vi "Main_Base.vi"() -> ()   [LabVIEW 2019]
uses:
  <vilib>/myRIO/Common/Instrument Driver Framework/myRIO v1.0/Encoder/typedefs/Encoder Signal Mode.ctl
  <vilib>/myRIO/Common/Instrument Driver Framework/myRIO v1.0/Encoder/typedefs/Encoder Configuration v1.0.ctl
  <vilib>/myRIO/Instrument Drivers/Onboard IO/Encoder/typedefs/Encoder Reference.ctl
  <vilib>/myRIO/Common/Instrument Driver Framework/Utilities/typedefs/myRIO Generic Hardware Reference.ctl
  <vilib>/myRIO/Common/Instrument Driver Framework/Utilities/typedefs/Hardware Version Enum.ctl
  <vilib>/myRIO/Common/Instrument Driver Framework/Utilities/typedefs/myRIO v1.0 Reference.ctl
  <vilib>/myRIO/Common/Instrument Driver Framework/Utilities/typedefs/Generic FPGA Reference.ctl
  <vilib>/myRIO/Common/Instrument Driver Framework/myRIO v1.0/Encoder/typedefs/Encoder Channels Enum.ctl
  <vilib>/userDefined/High Color/nirio_resource_hc.ctl
  <vilib>/myRIO/Instrument Drivers/Onboard IO/DIO/typedefs/DIO Reference.ctl
  <vilib>/myRIO/Common/Instrument Driver Framework/myRIO v1.0/DIO/typedefs/DIO Channels List.ctl
  <vilib>/myRIO/Common/Instrument Driver Framework/myRIO v1.0/DIO/typedefs/DIO Channels Enum.ctl
  <vilib>/myRIO/Instrument Drivers/Onboard IO/PWM/typedefs/PWM Reference.ctl
  <vilib>/myRIO/Common/Instrument Driver Framework/myRIO v1.0/PWM/typedefs/PWM Channels Enum.ctl
  <vilib>/myRIO/Instrument Drivers/Onboard IO/PWM/typedefs/PWM Configuration.ctl
  <vilib>/myRIO/Common/Instrument Driver Framework/myRIO v1.0/Encoder/vis/myRIO v1.1 Open Encoder.vi
  <vilib>/myRIO/Common/Instrument Driver Framework/myRIO v1.0/DIO/vis/myRIO v1.1 Open DIO.vi
  <vilib>/myRIO/Common/Instrument Driver Framework/myRIO v1.0/PWM/vis/myRIO v1.1 Open PWM.vi
  <vilib>/myRIO/Common/Instrument Driver Framework/Utilities/vis/Validate Channels.vi
  <vilib>/myRIO/Common/Instrument Driver Framework/myRIO v1.0/Encoder/vis/myRIO v1.0 Reserve Encoder.vi
  <vilib>/myRIO/Common/Instrument Driver Framework/myRIO v1.0/DIO/vis/myRIO v1.0 Reserve DIO.vi
  <vilib>/myRIO/Common/Instrument Driver Framework/myRIO v1.0/PWM/vis/myRIO v1.0 Reserve PWM.vi
  <vilib>/myRIO/Instrument Drivers/Onboard IO/PWM/vis/Set Duty Cycle and Frequency.vi
  <vilib>/myRIO/Common/Instrument Driver Framework/myRIO v1.0/Encoder/vis/myRIO v1.0 Close Encoder.vi
  <vilib>/myRIO/Common/Instrument Driver Framework/myRIO v1.0/DIO/vis/myRIO v1.0 Close DIO.vi
  <vilib>/myRIO/Common/Instrument Driver Framework/myRIO v1.0/PWM/vis/myRIO v1.0 Close PWM.vi
  <vilib>/myRIO/Common/Instrument Driver Framework/myRIO v1.0/Encoder/vis/myRIO v1.0 Build MUX Configuration Encoder.vi
  <vilib>/myRIO/Common/Instrument Driver Framework/myRIO v1.0/Resource Manager/vis/myRIO v1.0 Reserve Channel List.vi
  <vilib>/myRIO/Common/Instrument Driver Framework/myRIO v1.0/DIO/vis/myRIO v1.0 Build MUX Configuration DIO.vi
  <vilib>/myRIO/Common/Instrument Driver Framework/myRIO v1.0/PWM/vis/myRIO v1.0 Build MUX Configuration PWM.vi
  <vilib>/myRIO/Common/Instrument Driver Framework/myRIO v1.0/Encoder/vis/myRIO v1.0 Unreserve Encoder.vi
  <vilib>/myRIO/Common/Instrument Driver Framework/myRIO v1.0/DIO/vis/myRIO v1.0 Unreserve DIO.vi
  <vilib>/myRIO/Common/Instrument Driver Framework/myRIO v1.0/PWM/vis/myRIO v1.0 Unreserve PWM.vi
  <vilib>/myRIO/Common/Instrument Driver Framework/myRIO v1.0/Resource Manager/vis/myRIO v1.0 Create Configuration List.vi
  <vilib>/myRIO/Common/Instrument Driver Framework/myRIO v1.0/Resource Manager/vis/myRIO v1.0 Reserve Channel.vi
  <vilib>/myRIO/Common/Instrument Driver Framework/myRIO v1.0/Resource Manager/vis/myRIO v1.0 Unreserve Channel.vi
  <vilib>/myRIO/Common/Instrument Driver Framework/myRIO v1.0/Resource Manager/vis/myRIO v1.0 Unreserve Channel List.vi
  <vilib>/myRIO/Common/Instrument Driver Framework/myRIO v1.0/Resource Manager/vis/myRIO v1.0 Build Mutex Name.vi
  <vilib>/Utility/VariantDataType/GetNumericInfo.vi
  <vilib>/Utility/error.llb/Error Cluster From Error Code.vi
  <vilib>/myRIO/Common/Instrument Driver Framework/myRIO v1.0/myRIO v1.1 Open.vi
  <vilib>/myRIO/Common/Instrument Driver Framework/Utilities/vis/IO Manager.vi
  <vilib>/myRIO/Common/Instrument Driver Framework/Utilities/vis/Configuration Manager.vi
  <vilib>/myRIO/Common/Instrument Driver Framework/myRIO v1.0/Resource Manager/vis/myRIO v1.0 Configure IO.vi
  <vilib>/myRIO/Common/Instrument Driver Framework/myRIO v1.0/myRIO v1.0 Close.vi
  <vilib>/myRIO/Common/Instrument Driver Framework/myRIO v1.0/PWM/vis/myRIO v1.0 Write PWM.vi
  <vilib>/myRIO/Common/Instrument Driver Framework/myRIO v1.0/Encoder/vis/myRIO v1.0 Configure Encoder.vi
  <vilib>/myRIO/Common/Instrument Driver Framework/myRIO v1.0/Encoder/vis/myRIO v1.0 Enable Encoder.vi
  <vilib>/myRIO/Common/Instrument Driver Framework/myRIO v1.0/Encoder/vis/myRIO v1.0 Read Encoder.vi
  <vilib>/myRIO/Common/Instrument Driver Framework/myRIO v1.0/DIO/vis/myRIO v1.0 Write DIO.vi
  <vilib>/myRIO/Common/Instrument Driver Framework/myRIO v1.0/Encoder/vis/myRIO v1.0 Shutdown Encoder.vi
  <vilib>/myRIO/Common/Instrument Driver Framework/myRIO v1.0/DIO/vis/myRIO v1.0 Shutdown DIO.vi
  <vilib>/myRIO/Common/Instrument Driver Framework/myRIO v1.0/PWM/vis/myRIO v1.0 Shutdown PWM.vi
  <vilib>/myRIO/Instrument Drivers/Onboard IO/PWM/vis/myRIO PWM Open.xnode
  <vilib>/myRIO/Instrument Drivers/Onboard IO/DIO/vis/myRIO DIO Open.xnode
  <vilib>/myRIO/Instrument Drivers/Onboard IO/Encoder/vis/myRIO Encoder Open.xnode
  <vilib>/myRIO/Instrument Drivers/Onboard IO/PWM/PWM.lvlib
  <vilib>/myRIO/Instrument Drivers/Onboard IO/DIO/DIO.lvlib
  <vilib>/myRIO/Instrument Drivers/Onboard IO/Encoder/Encoder.lvlib
panel:
  out "Y":dbl
  out "X":dbl
  out "Theta":dbl
  out "Delta_theta":dbl
  out "Delta_s":dbl
  out "Delta_s_R":dbl
  out "Delta_s_L":dbl
  out "RPM_R":dbl
  out "RPM_L":dbl
  out "Delta_t_safe_ms":u32
  out "Delta_t_ms":u32
  out "Delta_N_R":i32
  out "Delta_N_L":i32
  out "Encoder_R_Count":i32
  out "Encoder_L_Count":i32
  in  "STOP_EMERGENCIA":bool
  in  "Duty (%)":dbl min=0.0 max=100.0 step=1.0
  in  "Comando":T1(ring)
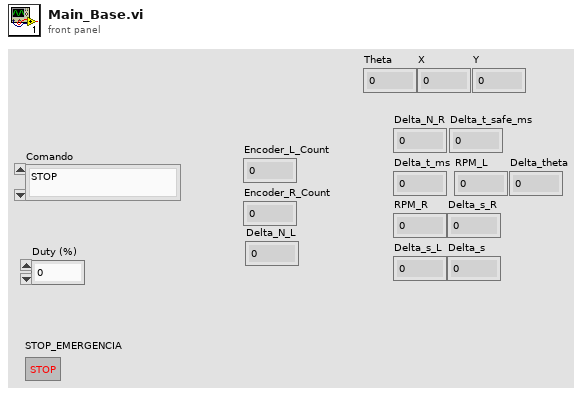
[diagram p1: front panel]
types:
  T1 = enum16{"STOP", "ADELANTE", "ATRÁS", "GIRO_IZQ", "GIRO_DER"}
  T2 = typedef "Encoder Signal Mode.ctl" = enum16{"Quadrature phase signal", "Step and direction signal"}
  T3 = typedef "Encoder.lvlib/Encoder Reference.ctl" = cluster{"myRIO Reference":T4, "Encoder Channels Enum":T8}
  T4 = typedef "myRIO Generic Hardware Reference.ctl" = cluster{"myRIO Model":T5, "myRIO Hardware Reference":T6}
  T5 = typedef "Hardware Version Enum.ctl" = enum16{"Unknown", "myRIO-1900", "myRIO-1950", "roboRIO", "NI ELVIS RIO CM", "ELVIS III"}
  T6 = typedef "myRIO v1.0 Reference.ctl" = cluster{"Generic FPGA Reference":T7, "Allow multiple opens":bool}
  T7 = typedef "Generic FPGA Reference.ctl" = refnum<k20>
  T8 = typedef "Encoder Channels Enum.ctl" = enum16{"Not Connected", "C/ENC0", "C/ENC1", "A/ENC", "A/ENC0", "A/ENC1", "A/ENC2", "A/ENC3", "A/ENC4", "A/ENC5", "A/ENC6", "A/ENC7", "A/ENC8", "A/ENC9", "B/ENC", "B/ENC0", "B/ENC1", "B/ENC2", "B/ENC3", "B/ENC4", "B/ENC5", "B/ENC6", "B/ENC7", "B/ENC8", "B/ENC9", "DIO/ENC0", "DIO/ENC1", "DIO/ENC2", "DIO/ENC3", "DIO/ENC4"}
  T9 = typedef "DIO.lvlib/DIO Reference.ctl" = cluster{"myRIO Reference":T4, "DIO Channels List":T10}
  T10 = typedef "DIO Channels List.ctl" = T11[]
  T11 = typedef "DIO Channels Enum.ctl" = enum16{"Not Connected", "C/DIO0", "C/DIO1", "C/DIO2", "C/DIO3", "C/DIO4", "C/DIO5", "C/DIO6", "C/DIO7", "A/DIO0", "A/DIO1", "A/DIO2", "A/DIO3", "A/DIO4", "A/DIO5", "A/DIO6", "A/DIO7", "A/DIO8", "A/DIO9", "A/DIO10", "A/DIO11", "A/DIO12", "A/DIO13", "A/DIO14", "A/DIO15", "A/DIO16", "A/DIO17", "A/DIO18", "A/DIO19", "B/DIO0", "B/DIO1", "B/DIO2", "B/DIO3", "B/DIO4", "B/DIO5", "B/DIO6", "B/DIO7", "B/DIO8", "B/DIO9", "B/DIO10", "B/DIO11", "B/DIO12", "B/DIO13", "B/DIO14", "B/DIO15", "B/DIO16", "B/DIO17", "B/DIO18", "B/DIO19", "LED0", "LED1", "LED2", "LED3", "Button0", "DIO/DIO0", "DIO/DIO1", "DIO/DIO2", "DIO/DIO3", "DIO/DIO4", "DIO/DIO5", "DIO/DIO6", "DIO/DIO7", "DIO/DIO8", "DIO/DIO9", "SPI/CS0", "SPI/CS1", "SPI/CS2", "SPI/CS3", "LED RADIO (Green)", "LED RADIO (Red)", "LED COMM (Green)", "LED COMM (Red)", "LED MODE (Green)", "LED MODE (Red)"}
  T12 = typedef "PWM.lvlib/PWM Reference.ctl" = cluster{"myRIO Reference":T4, "PWM Channels Enum":T13, "PWM Configuration":T14}
  T13 = typedef "PWM Channels Enum.ctl" = enum16{"Not Connected", "C/PWM0", "C/PWM1", "A/PWM0", "A/PWM1", "A/PWM2", "A/PWM3", "A/PWM4", "A/PWM5", "A/PWM6", "A/PWM7", "A/PWM8", "A/PWM9", "A/PWM10", "A/PWM11", "A/PWM12", "A/PWM13", "A/PWM14", "A/PWM15", "A/PWM16", "A/PWM17", "A/PWM18", "A/PWM19", "B/PWM0", "B/PWM1", "B/PWM2", "B/PWM3", "B/PWM4", "B/PWM5", "B/PWM6", "B/PWM7", "B/PWM8", "B/PWM9", "B/PWM10", "B/PWM11", "B/PWM12", "B/PWM13", "B/PWM14", "B/PWM15", "B/PWM16", "B/PWM17", "B/PWM18", "B/PWM19", "PWM/PWM0", "PWM/PWM1", "PWM/PWM2", "PWM/PWM3", "PWM/PWM4", "PWM/PWM5", "PWM/PWM6", "PWM/PWM7", "PWM/PWM8", "PWM/PWM9"}
  T14 = typedef "PWM.lvlib/PWM Configuration.ctl" = cluster{"Frequency":dbl, "Duty Cycle":dbl}
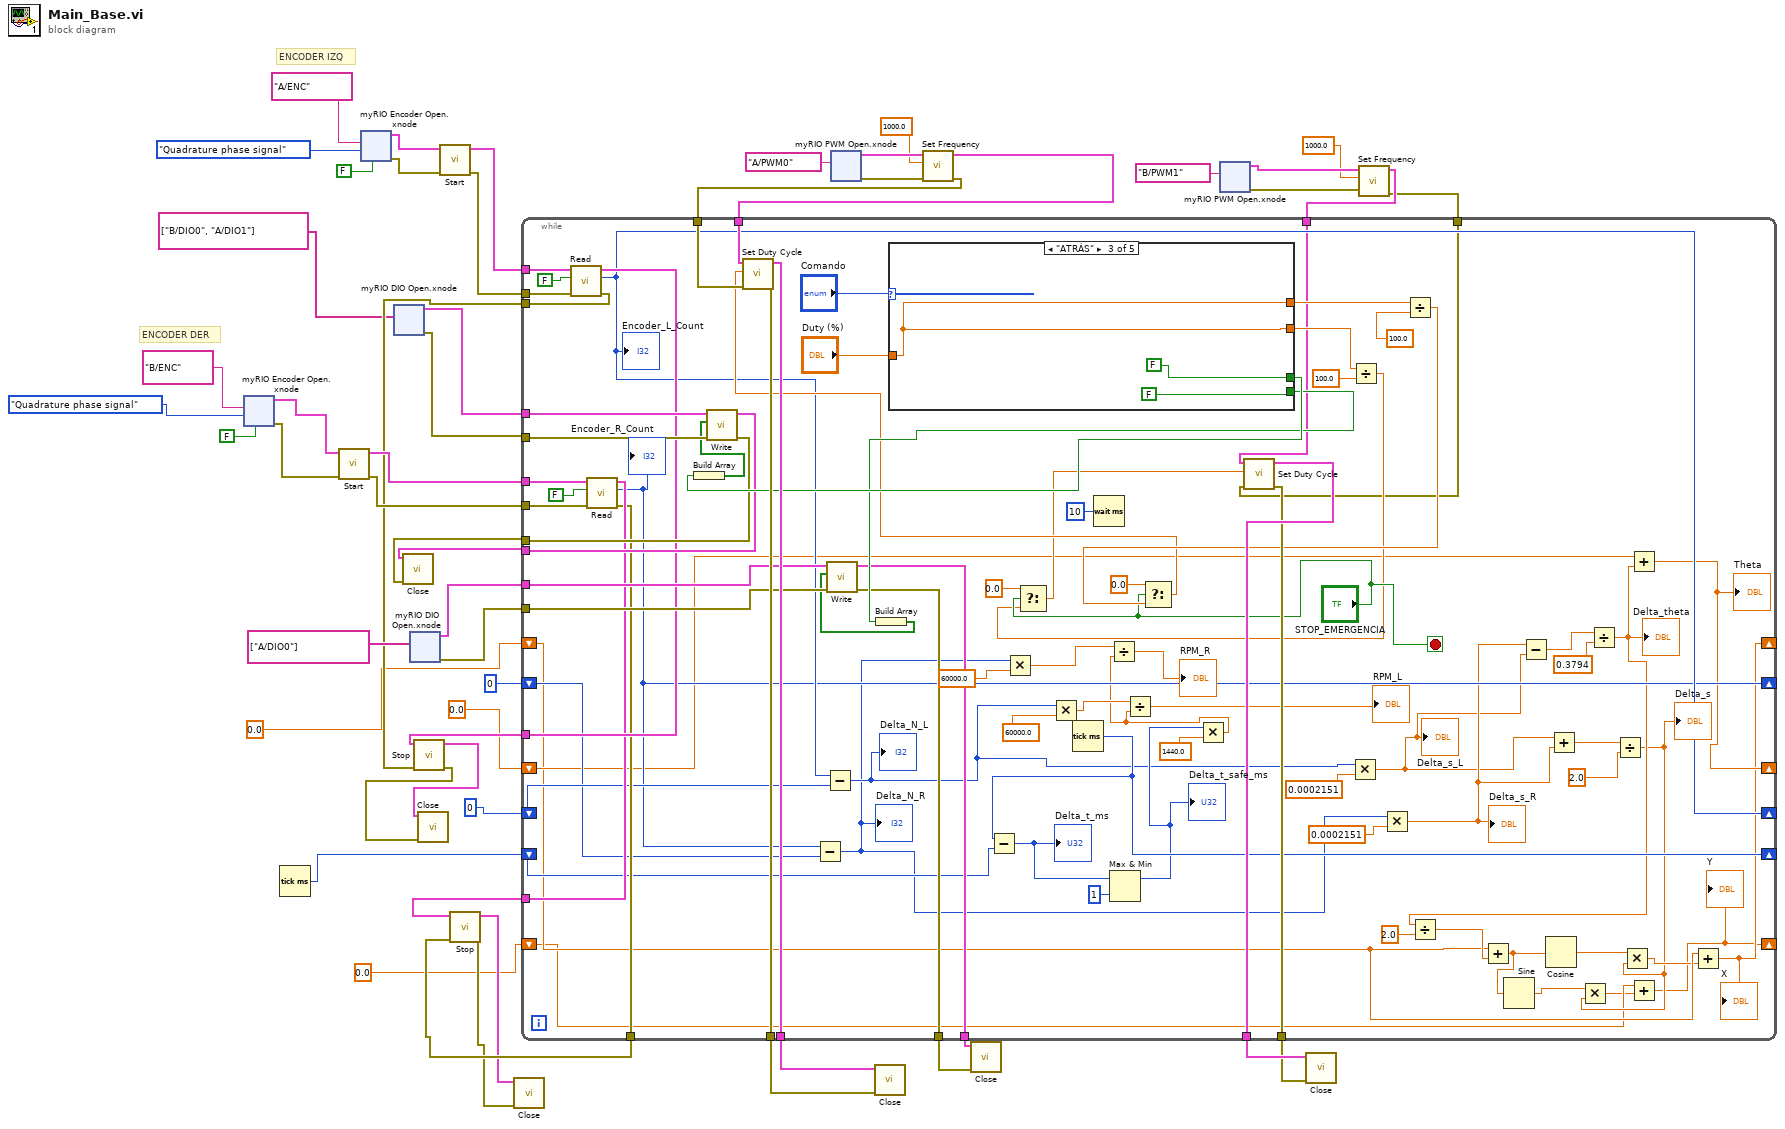
[diagram p0: block diagram]
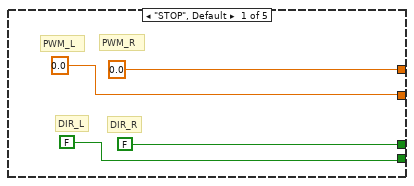
[diagram p2: hidden frame]
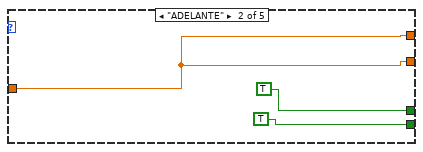
[diagram p3: hidden frame]
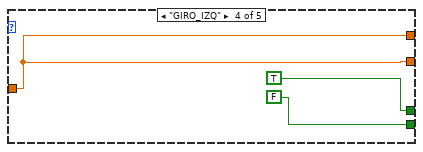
[diagram p4: hidden frame]
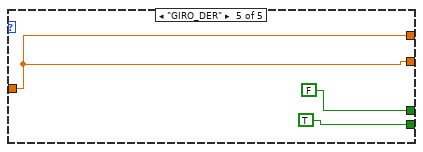
[diagram p5: hidden frame]
diagram:
  # "ENCODER DER"
  # "ENCODER IZQ"
  n1 = xnode "myRIO Encoder Open.xnode"("Channel Name"=tag "B/ENC", "Start Counter"=FALSE, "Encoder Signal Mode"=Encoder_Signal_Mode."Quadrature phase signal") -> ("error out"=w20:errorcluster, "Encoder Ref Out"=w21:T3)  [unwired: 2 in]
  n2 = Tick Count (ms)() -> (millisecond timer value=w7:u32)
  n3 = call <vilib>:"Start.vi"("error in (no error)"=w20, "Encoder Ref In"=w21) -> ("error out"=w18:errorcluster, "Encoder Ref Out"=w19:T3)  [unwired: 8 in]
  n4 = xnode "myRIO Encoder Open.xnode"("Channel Name"=tag "A/ENC", "Start Counter"=FALSE, "Encoder Signal Mode"=Encoder_Signal_Mode."Quadrature phase signal") -> ("error out"=w27:errorcluster, "Encoder Ref Out"=w28:T3)  [unwired: 2 in]
  n5 = xnode "myRIO DIO Open.xnode"("Channel Names"=tag[] ["B/DIO0", "A/DIO1"]) -> ("error out"=w39:errorcluster, "DIO Ref Out"=w40:T9)  [unwired: 2 in]
  n6 = xnode "myRIO DIO Open.xnode"("Channel Names"=tag[] ["A/DIO0"]) -> ("error out"=w34:errorcluster, "DIO Ref Out"=w35:T9)  [unwired: 2 in]
  n7 = call <vilib>:"Start.vi"("error in (no error)"=w27, "Encoder Ref In"=w28) -> ("error out"=w25:errorcluster, "Encoder Ref Out"=w26:T3)  [unwired: 8 in]
  n8 = xnode "myRIO PWM Open.xnode"("Channel Name"=tag "A/PWM0") -> ("error out"=w52:errorcluster, "PWM Ref Out"=w53:T12)  [unwired: 2 in]
  n9 = call <vilib>:"Set Frequency.vi"("error in (no error)"=w52, "Frequency [Hz]"=1000.0, "PWM Ref In"=w53) -> ("error out"=w49:errorcluster, "PWM Ref Out"=w50:T12)  [unwired: 6 in]
  n10 = xnode "myRIO PWM Open.xnode"("Channel Name"=tag "B/PWM1") -> ("error out"=w45:errorcluster, "PWM Ref Out"=w44:T12)  [unwired: 2 in]
  n11 = call <vilib>:"Set Frequency.vi"("error in (no error)"=w45, "Frequency [Hz]"=1000.0, "PWM Ref In"=w44) -> ("error out"=w1:errorcluster, "PWM Ref Out"=w2:T12)  [unwired: 6 in]
  n12 = while {
    tunnel: w50 -> [w133]
    tunnel: w49 -> [w132]
    tunnel: [w131] -> w48
    tunnel: [w130] -> w47
    tunnel: [w129] -> w42
    tunnel: [w128] -> w41
    tunnel: w40 -> [w127]
    tunnel: w39 -> [w126]
    tunnel: [w123] -> w38
    tunnel: [w122] -> w37
    tunnel: w35 -> [w121]
    tunnel: w34 -> [w120]
    tunnel: [w117] -> w33
    tunnel: [w116] -> w32
    tunnel: w26 -> [w108]
    tunnel: w25 -> [w107]
    tunnel: w19 -> [w105]
    tunnel: w18 -> [w104]
    tunnel: [w102] -> w17
    tunnel: [w101] -> w16
    tunnel: [w100] -> w13
    tunnel: [w99] -> w12
    shift-right: [w98] -> _
    shift-left: 0 ("Counter Value") -> [w97]
    shift-right: [w96] -> _
    shift-left: 0 ("Counter Value") -> [w95]
    shift-right: [w94] -> _
    shift-left: w7 -> [w93]
    shift-right: [w70] -> _
    shift-left: 0.0 -> [w71]
    shift-right: [w63] -> _
    shift-left: 0.0 -> [w65]
    shift-right: [w57] -> _
    shift-left: 0.0 -> [w59]
    tunnel: w2 -> [w56]
    tunnel: w1 -> [w55]
    stop <- "STOP_EMERGENCIA" stop-if-true
    n13 = call <vilib>:"Read.vi"("error in (no error)"=w107, "Reset Counter"=FALSE, "Encoder Ref In"=w108) -> ("error out"=w101:errorcluster, "Counter Value"=w98:i32, "Encoder Ref Out"=w102:T3)  [unwired: 4 in, 2 out]
    "Encoder_L_Count" <- w98
    n14 = call <vilib>:"Read.vi"("error in (no error)"=w104, "Reset Counter"=FALSE, "Encoder Ref In"=w105) -> ("error out"=w99:errorcluster, "Counter Value"=w96:i32, "Encoder Ref Out"=w100:T3)  [unwired: 4 in, 2 out]
    "Encoder_R_Count" <- w96
    n15 = Subtract(x=w96, y=w95) -> (x-y=w79:i32)
    "Delta_N_R" <- w79
    n16 = Subtract(x=w98, y=w97) -> (x-y=w81:i32)
    "Delta_N_L" <- w81
    n17 = case shown="\"ATRÁS\"" "Comando" {
      tunnel: [0.0 w147 w150 w153 w156] -> w134
      tunnel: [0.0 w147 w150 w153 w156] -> w136
      tunnel: [FALSE TRUE FALSE FALSE TRUE] -> w119
      tunnel: [FALSE TRUE FALSE TRUE FALSE] -> w124
      tunnel: "Duty (%)" -> [_ w147 w150 w153 w156]
      frame "STOP", Default {
        # "DIR_R"
        # "DIR_L"
        # "PWM_R"
        # "PWM_L"
      }
      frame "ADELANTE" {
      }
      frame "ATRÁS" {
      }
      frame "GIRO_IZQ" {
      }
      frame "GIRO_DER" {
      }
    }
    n18 = Build Array(w124) -> (w125:bool[])
    n19 = call <vilib>:"Write.vi"("error in (no error)"=w126, "Values"=w125, "DIO Ref In"=w127) -> ("error out"=w122:errorcluster, "DIO Ref Out"=w123:T9)  [unwired: 6 in]
    n20 = Build Array(w119) -> (w118:bool[])
    n21 = call <vilib>:"Write.vi"("error in (no error)"=w120, "Values"=w118, "DIO Ref In"=w121) -> ("error out"=w117:errorcluster, "DIO Ref Out"=w116:T9)  [unwired: 6 in]
    n22 = Multiply(x=w79, y=60000.0) -> (x*y=w84:dbl)
    n23 = Multiply(x=w81, y=60000.0) -> (x*y=w89:dbl)
    n24 = Tick Count (ms)() -> (millisecond timer value=w94:u32)
    n25 = Subtract(x=w94, y=w93) -> (x-y=w92:u32)
    "Delta_t_ms" <- w92
    n26 = Wait (ms)(milliseconds to wait=u32 10) -> ()  [unwired: 1 out]
    n27 = Max & Min(x=w92, y=u32 1) -> (max(x,y)=w88:u32)  [unwired: 1 out]
    "Delta_t_safe_ms" <- w88
    n28 = Multiply(x=w88, y=1440.0) -> (x*y=w83:dbl)
    n29 = Divide(x=w84, y=w83) -> (x/y=→"RPM_R":dbl)
    n30 = Divide(x=w89, y=w83) -> (x/y=→"RPM_L":dbl)
    n31 = Multiply(x=w81, y=0.0002151) -> (x*y=w74:dbl)
    "Delta_s_L" <- w74
    n32 = Divide(x=w134, y=100.0) -> (x/y=w110:dbl)
    n33 = Select(t=0.0, s="STOP_EMERGENCIA", f=w110) -> (s? t:f=w109:dbl)
    n34 = call <vilib>:"Set Duty Cycle.vi"("error in (no error)"=w55, "Duty Cycle"=w109, "PWM Ref In"=w56) -> ("error out"=w128:errorcluster, "PWM Ref Out"=w129:T12)  [unwired: 6 in]
    n35 = Multiply(x=w79, y=0.0002151) -> (x*y=w75:dbl)
    "Delta_s_R" <- w75
    n36 = Divide(x=w136, y=100.0) -> (x/y=w114:dbl)
    n37 = Select(t=0.0, s="STOP_EMERGENCIA", f=w114) -> (s? t:f=w113:dbl)
    n38 = call <vilib>:"Set Duty Cycle.vi"("error in (no error)"=w132, "Duty Cycle"=w113, "PWM Ref In"=w133) -> ("error out"=w130:errorcluster, "PWM Ref Out"=w131:T12)  [unwired: 6 in]
    n39 = Subtract(x=w75, y=w74) -> (x-y=w73:dbl)
    n40 = Add(x=w74, y=w75) -> (x+y=w77:dbl)
    n41 = Divide(x=w73, y=0.3794) -> (x/y=w69:dbl)
    "Delta_theta" <- w69
    n42 = Divide(x=w69, y=2.0) -> (x/y=w67:dbl)
    n43 = Add(x=w65, y=w67) -> (x+y=w62:dbl)
    n44 = Sine(x=w62) -> (sin(x)=w61:dbl)
    n45 = Cosine(x=w62) -> (cos(x)=w66:dbl)
    n46 = Divide(x=w77, y=2.0) -> (x/y=w60:dbl)
    "Delta_s" <- w60
    n47 = Multiply(x=w61, y=w60) -> (x*y=w58:dbl)
    n48 = Multiply(x=w66, y=w60) -> (x*y=w64:dbl)
    n49 = Add(x=w71, y=w69) -> (x+y=w70:dbl)
    "Theta" <- w70
    n50 = Add(x=w59, y=w58) -> (x+y=w57:dbl)
    "Y" <- w57
    n51 = Add(x=w65, y=w64) -> (x+y=w63:dbl)
    "X" <- w63
  }
  n52 = call <vilib>:"Close.vi"("error in (no error)"=w37, "DIO Ref In"=w38) -> ()  [unwired: 9 in, 1 out]
  n53 = call <vilib>:"Stop.vi"("error in (no error)"=w16, "Encoder Ref In"=w17) -> ("error out"=w14:errorcluster, "Encoder Ref Out"=w15:T3)  [unwired: 8 in]
  n54 = call <vilib>:"Close.vi"("error in (no error)"=w14, "Encoder Ref In"=w15) -> ()  [unwired: 9 in, 1 out]
  n55 = call <vilib>:"Stop.vi"("error in (no error)"=w12, "Encoder Ref In"=w13) -> ("error out"=w10:errorcluster, "Encoder Ref Out"=w11:T3)  [unwired: 8 in]
  n56 = call <vilib>:"Close.vi"("error in (no error)"=w10, "Encoder Ref In"=w11) -> ()  [unwired: 9 in, 1 out]
  n57 = call <vilib>:"Close.vi"("error in (no error)"=w47, "PWM Ref In"=w48) -> ()  [unwired: 9 in, 1 out]
  n58 = call <vilib>:"Close.vi"("error in (no error)"=w33, "DIO Ref In"=w32) -> ()  [unwired: 9 in, 1 out]
  n59 = call <vilib>:"Close.vi"("error in (no error)"=w41, "PWM Ref In"=w42) -> ()  [unwired: 9 in, 1 out]
